vi "Assert Not Equal Value and Type_Variant.vi"(4 "Execution time (s)":dbl=-1.0, 5 "Assert Only? (F)":bool, 6 "error code (1)":i32=1, 7 "Label":string, 8 "error in (no error)":errorcluster, 9 "Register with caller test (F)":bool, 10 "Actual":variant, 11 "Expected":variant) -> (0 "error out":errorcluster, 2 "Properties.Assert":refnum<class "Properties.Assert.lvclass">)   [LabVIEW 2020, in "Caraya.lvlib" / "Assert.lvclass"]
doc: "Generates an error if the input condition is not met.\n\nThis method compares the inputs.\nAsserts TRUE if either type or value of inputs differ.\nAsserts FALSE otherwise.\n\nex 1: Comparing two input integers of equal value and type will assert FALSE.\n\nex 2: Comparing two integer inputs of equal value but of different type representation (U8 and I32) will assert TRUE."
uses:
  Assert.lvclass
  Assert.lvclass/Assert.ctl
  <vilib>/Utility/VariantDataType/VariantType.lvlib
  <userlib>/_OpenG.lib/string/string.llb/openg_string.lvlib
  Properties/Properties.lvclass
  Properties.Assert/Properties.Assert.lvclass
  C:/Projects/caraya/src/classes/Properties/Properties.lvclass
  C:/Projects/caraya/src/classes/Properties.Assert/Properties.Assert.lvclass
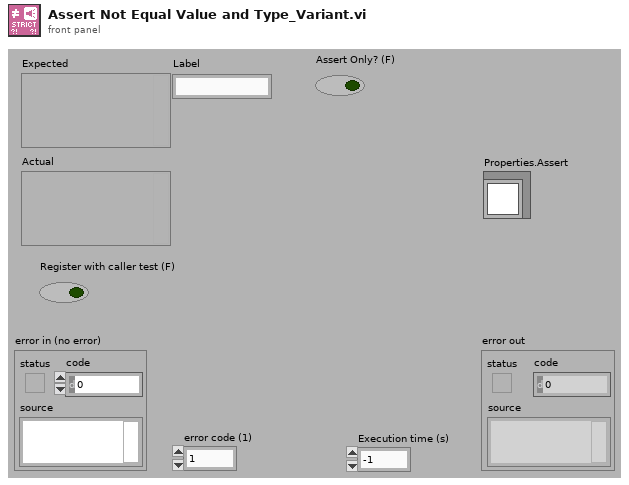
[diagram p1: front panel]
types:
  T1 = typedef "VariantType.lvlib/Type.ctl" = enum8{"Invalid Type", "Void", "I8", "I16", "I32", "I64", "U8", "U16", "U32", "U64", "Single Float", "Double Float", "Extended Float", "Single Complex", "Double Complex", "Extended Complex", "Enum U8", "Enum U16", "Enum U32", "Enum U64", "Single Float With Unit", "Double Float With Unit", "Extended Float With Unit", "Single Complex with Unit", "Double Complex with Unit", "Extended Complex with Unit", "Boolean", "String", "Path", "Picture", "Tag", "Array", "Cluster", "Variant", "LV Variant", "Waveform", "Timestamp", "Digital Waveform", "Digital Data", "ExpressData", "Refnum", "External Data", "VI", "Poly VI", "LabVIEW Class Instance", "Fixed Point"}
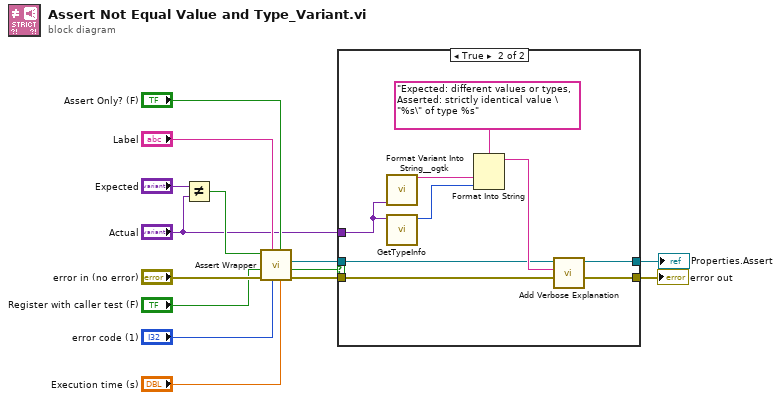
[diagram p0: block diagram]
diagram:
  n1 = Not Equal?(x="Expected", y="Actual") -> (x != y?=w12:bool)
  n2 = call "Assert Wrapper.vi"("Execution time (s)"="Execution time (s)", "Assert Only? (F)"="Assert Only? (F)", "error code (1)"="error code (1)", "Label"="Label", "error in (no error)"="error in (no error)", "Register with caller test (F)"="Register with caller test (F)", "Assert?"=w12) -> ("error out"=w8:errorcluster, "Verbose"=w4:bool, "Properties.Assert"=w2:refnum<class "Properties.Assert.lvclass">)  [unwired: 1 in, 1 out]
  n3 = case shown="True" w4 {
    tunnel: [w16 w20] -> w9
    tunnel: w8 -> [w16 w21]
    tunnel: "Actual" -> [_ w22]
    tunnel: w2 -> [w15 w18]
    tunnel: [w15 w17] -> w1
    frame False {
    }
    frame True {
      n4 = call <userlib>:"Format Variant Into String__ogtk.vi"("Variant"=w22) -> ("Output String"=w25:string)  [unwired: 13 in, 1 out]
      n5 = call <vilib>:"GetTypeInfo.vi"("Variant"=w22) -> ("Type Enum"=w23:T1)  [unwired: 6 in, 4 out]
      n6 = Format Into String(format string="Expected: different values or types, Asserted: strictly identical value \"%s\" of type %s" ("t"), w25, w23) -> (resulting string=w19:string)  [unwired: 2 in, 1 out]
      n7 = call "Add Verbose Explanation.vi"("error in (no error)"=w21, "Verbose Explanation"=w19, "Properties"=w18) -> ("error out"=w20:errorcluster, "Properties"=w17:refnum<class "Properties.Assert.lvclass">)  [unwired: 7 in]
    }
  }
  "error out" <- w9
  "Properties.Assert" <- w1
